vi "Main Editor UI.vi"() -> ()   [LabVIEW 2015, in "FPGA Module editor node.lvclass"]
doc: "This is the main view for configuration the behavior of a module in the DCAF standard editor."
uses:
  FPGA Module editor node.lvclass
  <vilib>/NI/Configuration Framework/Node/NodeRef.ctl
  <vilib>/NI/Configuration Framework/Node/NISE_CEF_Node.lvclass
  <vilib>/NI/AMC/Message Queue.ctl
  <vilib>/NI/AMC/Message.ctl
  <vilib>/NI/Tools/Keyed Array/KeyedArray.ctl
  <vilib>/NI/Configuration Framework/Node/UserEventRef.ctl
  <vilib>/NI/Configuration Framework/Controls/EventCluster.ctl
  <vilib>/NI/DCAF UI Toolkit/Controls/Configure.ctl
  <vilib>/NI/DCAF UI Toolkit/Controls/Add.ctl
  <vilib>/NI/DCAF UI Toolkit/Controls/Remove.ctl
  <vilib>/NI/Configuration Framework/Node/StopEvent.ctl
  <vilib>/NI/Configuration Framework/Node/RefreshUIEvent.ctl
  <vilib>/NI/Configuration Framework/Node/CacheState.ctl
  <vilib>/NI/Configuration Framework/Node/NodeChangeEvent.ctl
  <vilib>/NI/Tag Bus/tag/Data Type.ctl
  Permissions Enum.ctl
  <vilib>/NI/DCAF/Tag Editor Core/Table API/Available Tag Menu/channel action event.ctl
  <vilib>/NI/DCAF/Tag Editor Core/Table API/Available Tag Menu/dialog output action.ctl
  <vilib>/NI/Tag Bus Module Framework/channel/TBM channel.lvclass
  <vilib>/NI/Tag Bus/tag/tag descriptor.lvclass
  <vilib>/NI/DCAF/Tag Editor Core/Table API/Table Manager/Call Back Ref Type Def.ctl
  <vilib>/NI/DCAF/Tag Editor Core/Configuration Editor/Classes/Engine Parent/Engine Parent Editor Node.lvclass
  <vilib>/NI/DCAF/Tag Editor Core/Configuration Editor/Classes/Module editor node/module editor node.lvclass
  <vilib>/userdefined/High Color/nirio_resource_hc.ctl
  <vilib>/NI/DCAF/Tag Editor Core/Table API/Table Manager/references.ctl
  <vilib>/Utility/miscctls.llb/LVPositionTypeDef.ctl
  <vilib>/NI/DCAF/Tag Editor Core/Table API/Listbox/Multi Column Listbox.lvclass
  <vilib>/NI/Configuration Framework/NISE_CEF_TreeControl.lvlib
  <vilib>/NI/Tools/Keyed Array/Tools_KeyedArray.lvlib
  <vilib>/NI/AMC/AMC.lvlib
  <vilib>/NI/DCAF/Tag Editor Core/Table API/Table Manager.lvlib
  <vilib>/NI/DCAF/Tag Editor Core/Table API/Table Manager/Table Manager.lvclass
  <vilib>/NI/DCAF UI Toolkit/Controls/DCAF UI Elements.lvlib
panel:
  in  "user event out":refnum<user-event>
  in  "Permissions":T1
  in  "data type":T2
  in  "node change":T3
  in  "cache state":T4
  in  "refresh UI":T5
  in  "stop event":T6
  in  "Tab Control":enum32{"Channel Configuration"}(tab)
  in  "Import Channels":bool
  in  "Remove Button":T7
  in  "Add Button":T8
  in  "Table":i32(listbox)
  in  "settings":T9
  in  "RIO Device":T10
  in  "user event":T11
  in  "main queue":T12
  in  "node ref":T13
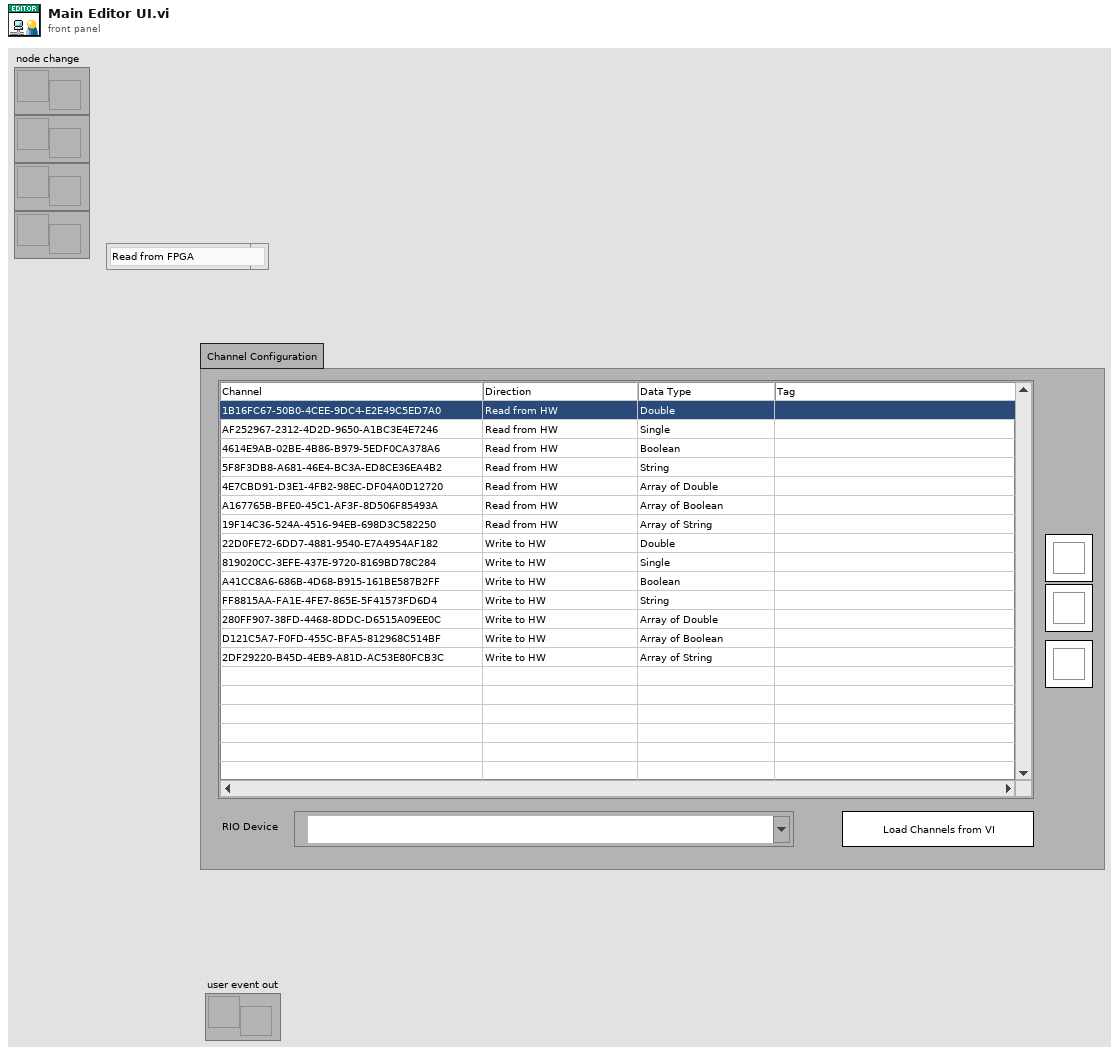
[diagram p1: front panel]
types:
  T1 = typedef "FPGA Module editor node.lvclass/Permissions Enum.ctl" = enum16{"Read from FPGA", "Write to FPGA"}
  T2 = typedef "tag bus.lvlib/tag descriptor.lvclass/Data Type.ctl" = enum16{"Double", "Single", "I64", "I32", "I16", "I8", "U64", "U32", "U16", "U8", "Boolean", "String", "Array of Double", "Array of Single", "Array of I64", "Array of I32", "Array of I16", "Array of I8", "Array of U64", "Array of U32", "Array of U16", "Array of U8", "Array of Boolean", "Array of String"}
  T3 = typedef "NISE_CEF_Node.lvclass/NodeChangeEvent.ctl" = refnum<user-event>
  T4 = typedef "NISE_CEF_Node.lvclass/CacheState.ctl" = refnum<user-event>
  T5 = typedef "NISE_CEF_Node.lvclass/RefreshUIEvent.ctl" = refnum<user-event>
  T6 = typedef "NISE_CEF_Node.lvclass/StopEvent.ctl" = refnum<user-event>
  T7 = typedef "DCAF UI Elements.lvlib/Remove.ctl" = bool
  T8 = typedef "DCAF UI Elements.lvlib/Add.ctl" = bool
  T9 = typedef "DCAF UI Elements.lvlib/Configure.ctl" = bool
  T10 = typedef "nirio_resource_hc.ctl" = tag
  T11 = typedef "NISE_CEF_Node.lvclass/UserEventRef.ctl" = refnum<user-event>
  T12 = typedef "AMC.lvlib/Message Queue.ctl" = refnum<queue>
  T13 = typedef "NISE_CEF_Node.lvclass/NodeRef.ctl" = refnum<data-value>
  T14 = typedef "Table Manager.lvlib/Table Manager.lvclass/references.ctl" = cluster{"stop event":T6, "refresh UI":T5, "cache state":T4, "node change":T3, "user event out":refnum<user-event>, "main queue":T12, "user event":T11}
  T15 = typedef "LVPositionTypeDef.ctl" = cluster{"Left":i32, "Top":i32}
  T16 = typedef "Table Manager.lvlib/Table Manager.lvclass/object ref.ctl" = cluster{"engine":refnum<data-value>, "Node Ref":refnum<data-value>}
  T17 = typedef "Table Manager.lvlib/Column.lvclass/Column Descriptor.ctl" = cluster{"name":string, "caption":string, "Column Type":T18, "Params":string, "AutoSizeMode":i32, "FillWeight":sgl, "MinWidth":u32, "tooltip":string, "Enum Reference":refnum<vi>, "Channel suffix":string, "Read Only":bool, "Call Back VI":T19, "DT Dependency":i32, "name dependency":i32, "data type":T2, "Custom Column":refnum<class "Column.lvclass">}
  T18 = typedef "Table Manager.lvlib/Column.lvclass/Column Type.ctl" = enum16{"String", "Mapping", "Enum", "Custom"}
  T19 = typedef "Table Manager.lvlib/Table Manager.lvclass/Call Back Ref Type Def.ctl" = refnum<vi>
  T20 = typedef "Table Manager.lvlib/Table Manager.lvclass/Table Events.ctl" = cluster{"Menu Selection":refnum<user-event>}
  T21 = enum8{"Enabled", "Disabled", "Disabled and Grayed Out"}
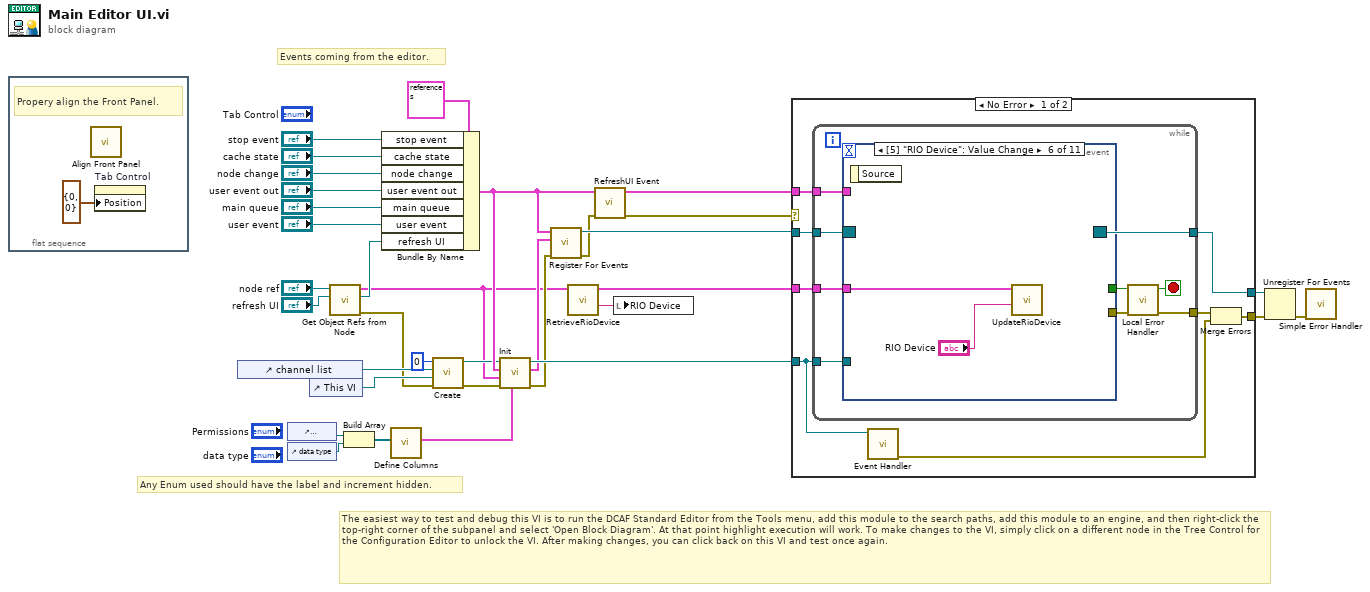
[diagram p0: block diagram]
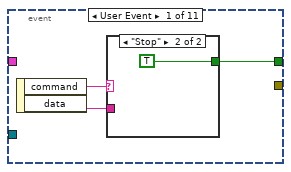
[diagram p2: hidden frame]
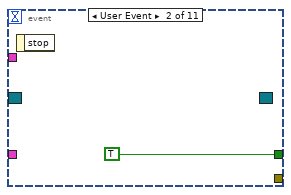
[diagram p4: hidden frame]
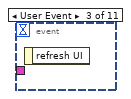
[diagram p5: hidden frame]
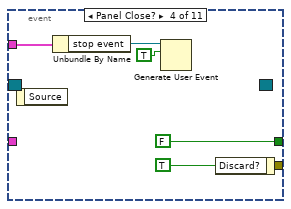
[diagram p6: hidden frame]
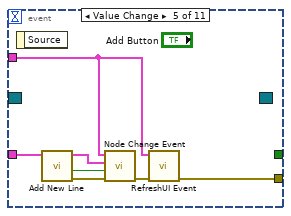
[diagram p7: hidden frame]
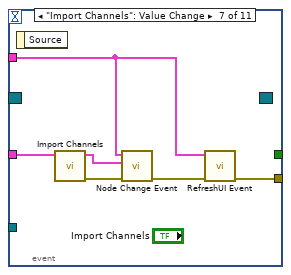
[diagram p8: hidden frame]
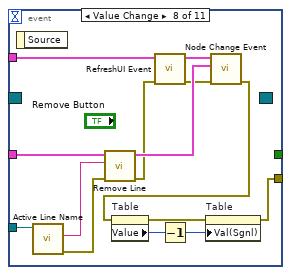
[diagram p9: hidden frame]
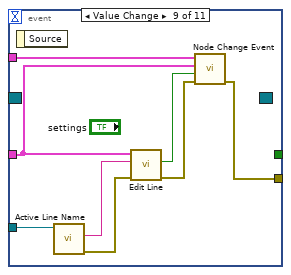
[diagram p10: hidden frame]
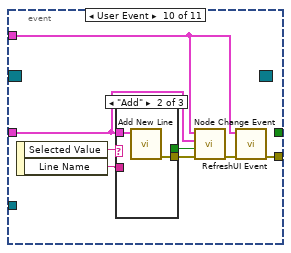
[diagram p11: hidden frame]
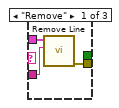
[diagram p12: hidden frame]
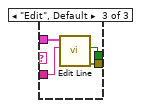
[diagram p13: hidden frame]
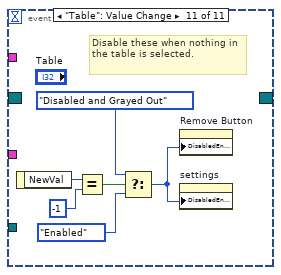
[diagram p14: hidden frame]
diagram:
  # "The easiest way to test and debug this VI is to run the DCAF Standard Editor from the Tools menu, add this module to the search paths, add this module to an engine, and then right-click the top-right corner of the subpanel and select 'Open Block Diagram'. At that point highlight execution will work. To make changes to the VI, simply click on a different node in the Tree Control for the Configuration Editor to unlock the VI. After making changes, you can click back on this VI and test once again."
  # "Any Enum used should have the label and increment hidden."
  # "Events coming from the editor."
  n1 = flat-sequence {
    frame #0 {
      # "Propery align the Front Panel."
      n2 = call <vilib>:"Align Front Panel.vi"() -> ()  [unwired: 10 in, 2 out]
      n3 = property on="Tab Control" class="TabCtl (strict)"("Position"=T15 {"Left"=0, "Top"=0}) -> ()  [unwired: 2 in, 2 out]
    }
  }
  n4 = control-ref of="channel list"() -> (w11:refnum<vi>)
  n5 = control-ref of="Permissions"() -> (w20:refnum<vi>)
  n6 = control-ref of="data type"() -> (w19:refnum<vi>)
  n7 = control-ref of="This VI"() -> (w9:refnum<vi>)
  n8 = call "Get Object Refs from Node.vi"("Refresh UI"="refresh UI", "Data Value Reference in"="node ref") -> ("error out"=w6:errorcluster, "Refresh UI out"=w4:T5, "References"=w3:T16)  [unwired: 7 in]
  n9 = Build Array(w20, w19) -> (w18:refnum<vi>[])
  n10 = Bundle By Name(cluster=T14 {"stop event"=refnum, "refresh UI"=refnum, "cache state"=refnum, "node change"=refnum, "user event out"=refnum, "main queue"=refnum, "user event"=refnum} ("References"), "stop event"="stop event", "cache state"="cache state", "node change"="node change", "user event out"="user event out", "main queue"="main queue", "user event"="user event", "refresh UI"=w4) -> (w21:T14)
  n11 = call "Define Columns.vi"("Enum Array"=w18) -> ("Column Definition"=w23:T17[])  [unwired: 10 in]
  n12 = call <vilib>:"Create.vi"("error in (no error)"=w6, "Top VI"=w9, "Listbox"=w11, "Index"=0) -> ("error out"=w7:errorcluster, "reference out"=w8:refnum<class "Multi Column Listbox.lvclass">)  [unwired: 6 in]
  n13 = call-dynamic "Init.vi"("Column Descriptors"=w23, "error in (no error)"=w7, "Node object refs"=w3, "Event References"=w21, "Multi Column Listbox in"=w8) -> ("error out"=w13:errorcluster, "Table Events"=w12:T20, "Multi Column Listbox out"=w17:refnum<class "Multi Column Listbox.lvclass">)  [unwired: 4 in]
  n14 = call "Register For Events.vi"("error in"=w13, "Table Events"=w12, "References"=w21) -> ("error out"=w15:errorcluster, "Event Registration Refnum"=w24:refnum<event-registration>)  [unwired: 7 in]
  n15 = call "RetrieveRioDevice.vi"("References"=w3) -> ("RIO Device"=w2:T10, "References out"=w1:T16)  [unwired: 8 in, 1 out]
  n16 = call "RefreshUI Event.vi"("error in (no error)"=w15, "References in"=w21) -> ("error out"=w14:errorcluster, "References out"=w22:T14)  [unwired: 8 in]
  n17 = local write "RIO Device"(w2) -> ()
  n18 = case shown="No Error" w14 {
    selector: w14 -> [_ w122]
    tunnel: w24 -> [w43 w121]
    tunnel: [w42 w121] -> w34
    tunnel: [w36 w122] -> w33
    tunnel: w22 -> [w41 _]
    tunnel: w1 -> [w40 _]
    tunnel: w17 -> [w39 _]
    frame No Error {
      n19 = while {
        tunnel: w43 -> [w52]
        tunnel: [w51] -> w42
        tunnel: [w48] -> w37
        tunnel: w41 -> [w46]
        tunnel: w40 -> [w45]
        tunnel: w39 -> [w44]
        stop <- w50 stop-if-true
        n20 = event shown="[5] \"RIO Device\": Value Change" {
          selector: w52 -> [_ _ _ _ _ _ _ _ _ _ _]
          dyn-events: [_ _ _ _ _ _ _ _ _ _ _] -> w51
          timeout: _ -> [_ _ _ _ _ _ _ _ _ _ _]
          tunnel: [w55 TRUE _ FALSE _ _ _ _ _ _ _] -> w49
          tunnel: [_ _ _ _ w63 _ w75 w78 w95 w103 _] -> w47
          tunnel: w46 -> [_ _ _ w59 w67 _ w72 w89 w97 w99 _]
          tunnel: w45 -> [_ _ _ _ w68 w70 w76 w88 w93 w100 _]
          tunnel: w44 -> [_ _ _ _ _ _ _ w84 w94 _ _]
          event User Event {
            n21 = event-data() -> ("command"=w54:string, "data"=w53:string)  [unwired: 1 in]
            n22 = case shown="\"Stop\"" w54 {
              tunnel: [_ TRUE] -> w55
              tunnel: w53 -> [_ _]
              frame Default {
              }
              frame "Stop" {
              }
            }
          }
          event User Event {
            n23 = event-data() -> ()  [unwired: 1 in, 1 out]
          }
          event User Event {
            n24 = event-data() -> ()  [unwired: 1 in, 1 out]
          }
          event Panel Close? {
            n25 = event-data() -> ()  [unwired: 1 in, 1 out]
            n26 = Unbundle By Name(w59) -> ("stop event"=w58:T6)
            n27 = Generate User Event(user event=w58, event data cluster=TRUE ("event data")) -> ()  [unwired: 2 in, 2 out]
            n28 = event-data("Discard?"=TRUE) -> ()  [unwired: 1 in, 1 out]
          }
          event Value Change {
            n29 = event-data() -> ()  [unwired: 1 in, 1 out]
            n30 = call "Add New Line.vi"("objects"=w68) -> ("error out"=w66:errorcluster, "success"=w64:bool)  [unwired: 8 in, 1 out]
            n31 = call "Node Change Event.vi"("error in (no error)"=w66, "Send (T)"=w64, "objects"=w68, "References in"=w67) -> ("error out"=w65:errorcluster)  [unwired: 7 in]
            n32 = call "RefreshUI Event.vi"("error in (no error)"=w65, "References in"=w67) -> ("error out"=w63:errorcluster)  [unwired: 8 in, 1 out]
          }
          event Value Change {
            n33 = event-data() -> ()  [unwired: 1 in, 1 out]
            n34 = call "UpdateRioDevice.vi"("RIO Device"="RIO Device", "References"=w70) -> ()  [unwired: 9 in, 1 out]
          }
          event "Import Channels": Value Change {
            n35 = event-data() -> ()  [unwired: 1 in, 1 out]
            n36 = call "Import Channels.vi"("Objects in"=w76) -> ("error out"=w74:errorcluster, "Objects out"=w71:T16)  [unwired: 9 in]
            n37 = call "Node Change Event.vi"("error in (no error)"=w74, "objects"=w71, "References in"=w72) -> ("error out"=w73:errorcluster)  [unwired: 8 in]
            n38 = call "RefreshUI Event.vi"("error in (no error)"=w73, "References in"=w72) -> ("error out"=w75:errorcluster)  [unwired: 8 in, 1 out]
          }
          event Value Change {
            n39 = event-data() -> ()  [unwired: 1 in, 1 out]
            n40 = call-dynamic "Active Line Name.vi"("Multi Column Listbox in"=w84) -> ("error out"=w82:errorcluster, "Active Line Name"=w83:string)  [unwired: 8 in, 1 out]
            n41 = call "Remove Line.vi"("error in"=w82, "Active Line Name"=w83, "Objects"=w88) -> ("error out"=w85:errorcluster)  [unwired: 8 in]
            n42 = call "RefreshUI Event.vi"("error in (no error)"=w85, "References in"=w89) -> ("error out"=w87:errorcluster, "References out"=w86:T14)  [unwired: 8 in]
            n43 = call "Node Change Event.vi"("error in (no error)"=w87, "objects"=w88, "References in"=w86) -> ("error out"=w79:errorcluster)  [unwired: 8 in]
            n44 = property on="Table" class="MCListbox (strict)"(error in=w79) -> (error out=w77:errorcluster, "Value"=w80:i32)  [unwired: 1 in, 1 out]
            n45 = Decrement(x=w80) -> (x-1=w81:i32)
            n46 = property on="Table" class="MCListbox (strict)"(error in=w77, "Val(Sgnl)"=w81) -> (error out=w78:errorcluster)  [unwired: 1 in, 1 out]
          }
          event Value Change {
            n47 = event-data() -> ()  [unwired: 1 in, 1 out]
            n48 = call-dynamic "Active Line Name.vi"("Multi Column Listbox in"=w94) -> ("error out"=w91:errorcluster, "Active Line Name"=w92:string)  [unwired: 8 in, 1 out]
            n49 = call "Edit Line.vi"("error in"=w91, "Line Name"=w92, "References"=w93) -> ("error out"=w96:errorcluster, "change?"=w90:bool)  [unwired: 7 in]
            n50 = call "Node Change Event.vi"("error in (no error)"=w96, "Send (T)"=w90, "objects"=w93, "References in"=w97) -> ("error out"=w95:errorcluster)  [unwired: 7 in]
          }
          event User Event {
            n51 = event-data() -> ("Selected Value"=w105:string, "Line Name"=w102:string)  [unwired: 1 in]
            n52 = case shown="\"Add\"" w105 {
              tunnel: w102 -> [w108 _ w114]
              tunnel: w100 -> [w107 w110 w113]
              tunnel: [w106 w109 w112] -> w101
              tunnel: [_ _ w111] -> w98
              frame "Remove" {
                n53 = call "Remove Line.vi"("Active Line Name"=w108, "Objects"=w107) -> ("error out"=w106:errorcluster)  [unwired: 9 in]
              }
              frame "Add" {
                n54 = call "Add New Line.vi"("objects"=w110) -> ("error out"=w109:errorcluster)  [unwired: 8 in, 2 out]
              }
              frame "Edit", Default {
                n55 = call "Edit Line.vi"("Line Name"=w114, "References"=w113) -> ("error out"=w112:errorcluster, "change?"=w111:bool)  [unwired: 8 in]
              }
            }
            n56 = call "Node Change Event.vi"("error in (no error)"=w101, "Send (T)"=w98, "objects"=w100, "References in"=w99) -> ("error out"=w104:errorcluster)  [unwired: 7 in]
            n57 = call "RefreshUI Event.vi"("error in (no error)"=w104, "References in"=w99) -> ("error out"=w103:errorcluster)  [unwired: 8 in, 1 out]
          }
          event "Table": Value Change {
            # "Disable these when nothing in the table is selected."
            n58 = event-data() -> ("NewVal"=w120:i32)  [unwired: 1 in]
            n59 = Equal?(x=w120, y=-1) -> (x = y?=w118:bool)
            n60 = Select(t=T21."Disabled and Grayed Out" ("Disabled"), s=w118, f=T21."Enabled") -> (s? t:f=w116:T21)
            n61 = property on="Remove Button" class="Bool"("DisabledEnum"=w116) -> ()  [unwired: 2 in, 2 out]
            n62 = property on="settings" class="Bool"("DisabledEnum"=w116) -> ()  [unwired: 2 in, 2 out]
          }
        }
        n63 = call "Local Error Handler.vi"("error in"=w47, "Stop in"=w49) -> ("error out"=w48:errorcluster, "Stop out"=w50:bool)  [unwired: 8 in]
      }
      n64 = call-dynamic "Event Handler.vi"("Listbox in"=w39) -> ("error out"=w38:errorcluster)  [unwired: 9 in, 1 out]
      n65 = Merge Errors(w37, w38) -> (w36:errorcluster)
    }
    frame Error {
    }
  }
  n66 = Unregister For Events(event registration refnum=w34, error in=w33) -> (error out=w32:errorcluster)
  n67 = call <vilib>:"Simple Error Handler.vi"("error in (no error)"=w32) -> ()  [unwired: 4 in, 5 out]
